vi "regexINISectionContent.vi"(8 "error in (no error)":errorcluster, 9 "Section Content":string, 10 "Section Name":string) -> (0 "error out":errorcluster, 1 "KVPs":cluster{"key":string, "value":string}[](array[cluster]), 2 "Section Name dup":string, 4 "Comments":string[](array[string]))   [LabVIEW 2013, in "CfgManager.Text.lvlib" / "ConfigManager.Text.INI.lvclass"]
uses:
  ConfigManager.Text.INI.lvclass
  <vilib>/regexp/Match Regular Expression.xnode
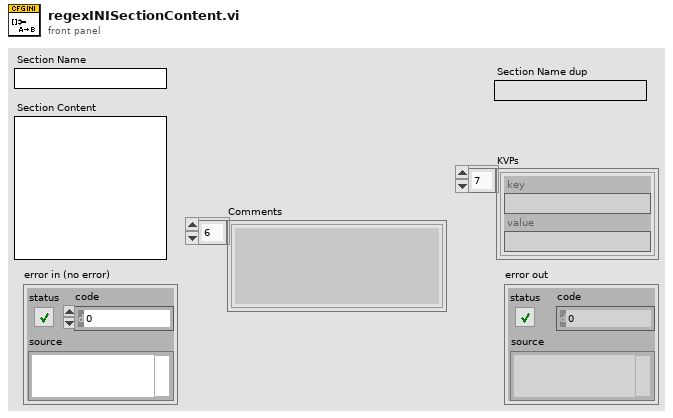
[diagram p1: front panel]
types:
  T1 = cluster{"trimmed string":string, "before match":string}
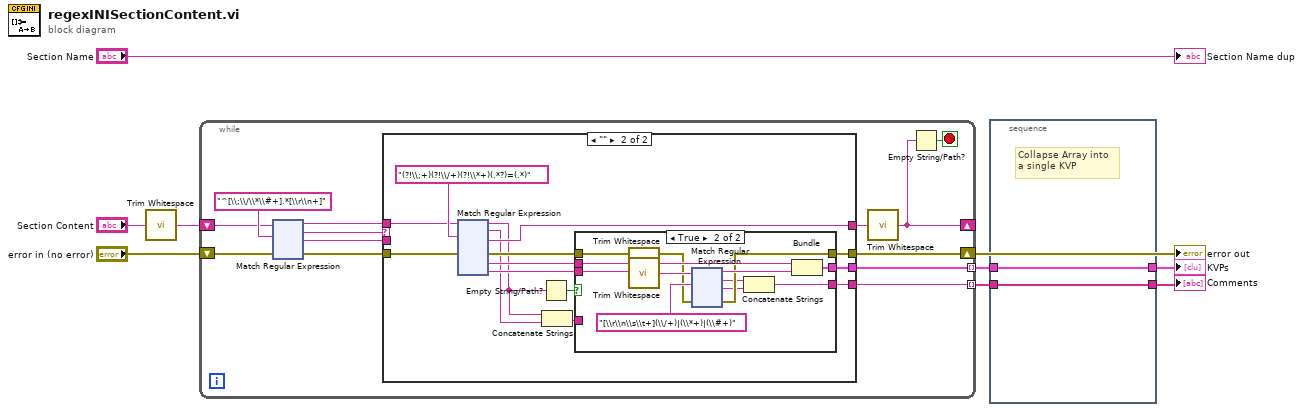
[diagram p0: block diagram]
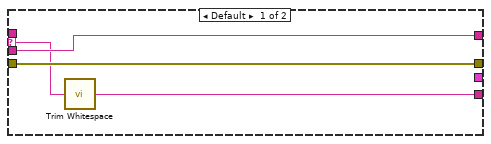
[diagram p2: hidden frame]
diagram:
  n1 = call <vilib>:"Trim Whitespace.vi"("string"="Section Content") -> ("trimmed string"=w5:string)  [unwired: 1 in]
  n2 = while {
    shift-right: [w19] -> _
    shift-left: w5 -> [w10]
    tunnel: [w22] -> w4 mode=indexing
    shift-right: [w18] -> w7
    shift-left: "error in (no error)" -> [w15]
    tunnel: [w17] -> w3 mode=indexing
    stop <- w21 stop-if-true
    n3 = xnode "Match Regular Expression"("input string"=w10, "regular expression"="^[\\;\\/\\*\\#+].*[\\r\\n+]" ("input string"), "error in"=w15) -> ("before match"=w11:string, "whole match"=w12:string, "after match"=w13:string, "error out"=w14:errorcluster)  [unwired: 3 in, 1 out]
    n4 = case shown="\"\"" w12 {
      selector: w12 -> [w24 _]
      tunnel: [_ w37] -> w22
      tunnel: [w26 w36] -> w20
      tunnel: [w25 w34] -> w18
      tunnel: [w23 w32] -> w17
      tunnel: w13 -> [w26 _]
      tunnel: w14 -> [w25 w28]
      tunnel: w11 -> [_ w27]
      frame Default {
        n5 = call <vilib>:"Trim Whitespace.vi"("string"=w24) -> ("trimmed string"=w23:string)  [unwired: 1 in]
      }
      frame "" {
        n6 = xnode "Match Regular Expression"("input string"=w27, "regular expression"="(?!\\;+)(?!\\/+)(?!\\*+)(.*?)=(.*)" ("input string"), "error in"=w28) -> ("before match"=w31:string, "whole match"=w30:string, "after match"=w36:string, "error out"=w35:errorcluster, "submatch 1"=w39:string, "submatch 2"=w38:string)  [unwired: 3 in, 1 out]
        n7 = Empty String/Path?(string/path=w31) -> (empty?=w33:bool)
        n8 = Concatenate Strings(w31, w30) -> (w29:string)
        n9 = case shown="True" w33 {
          tunnel: w39 -> [_ w54]
          tunnel: w38 -> [_ w53]
          tunnel: [_ w52] -> w37
          tunnel: w35 -> [w42 w47]
          tunnel: [w42 w46] -> w34
          tunnel: [w41 w43] -> w32
          tunnel: w29 -> [w41 _]
          frame False {
          }
          frame True {
            n10 = call <vilib>:"Trim Whitespace.vi"("string"=w54) -> ("trimmed string"=w51:string)  [unwired: 1 in]
            n11 = call <vilib>:"Trim Whitespace.vi"("string"=w53) -> ("trimmed string"=w50:string)  [unwired: 1 in]
            n12 = xnode "Match Regular Expression"("input string"=w50, "regular expression"="[\\r\\n\\s\\t+](\\/+)|(\\*+)|(\\#+)" ("input string"), "error in"=w47) -> ("before match"=w49:string, "whole match"=w45:string, "after match"=w44:string, "error out"=w46:errorcluster)  [unwired: 3 in, 1 out]
            n13 = Concatenate Strings(w45, w44) -> (w43:string)
            n14 = Bundle("trimmed string"=w51, "before match"=w49) -> (w52:T1)  [unwired: 1 in]
          }
        }
      }
    }
    n15 = call <vilib>:"Trim Whitespace.vi"("string"=w20) -> ("trimmed string"=w19:string)  [unwired: 1 in]
    n16 = Empty String/Path?(string/path=w19) -> (empty?=w21:bool)
  }
  "error out" <- w7
  n17 = stacked-sequence {
    tunnel: w4 -> [w401]
    tunnel: w3 -> [w400]
    tunnel: [w401] -> w2
    tunnel: [w400] -> w1
    frame #0 {
      # "Collapse Array into\na single KVP"
    }
  }
  "KVPs" <- w2
  "Comments" <- w1
  "Section Name dup" <- "Section Name"
